vi "Action-x_control_excel.vi"() -> ()   [LabVIEW 2018, in "Report_modify.lvlib"]
uses:
  Report_modify.lvlib
panel:
  out "数据":string[][](array[string])
  in  "Excel._Worksheet":refnum<k7>
  in  "Excel._Application":refnum<k7>
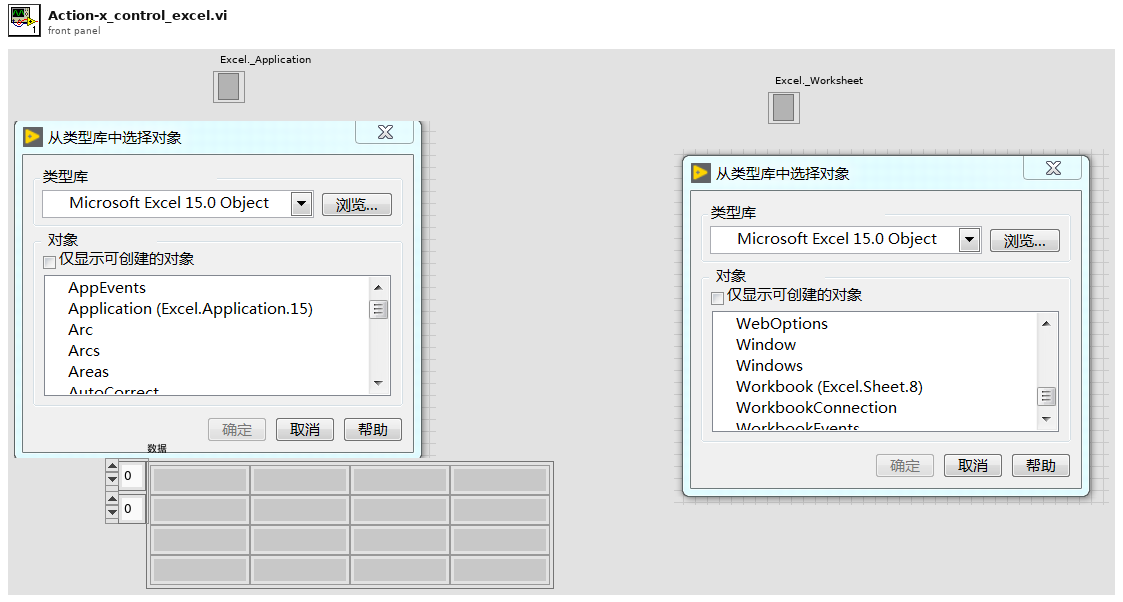
[diagram p1: front panel]
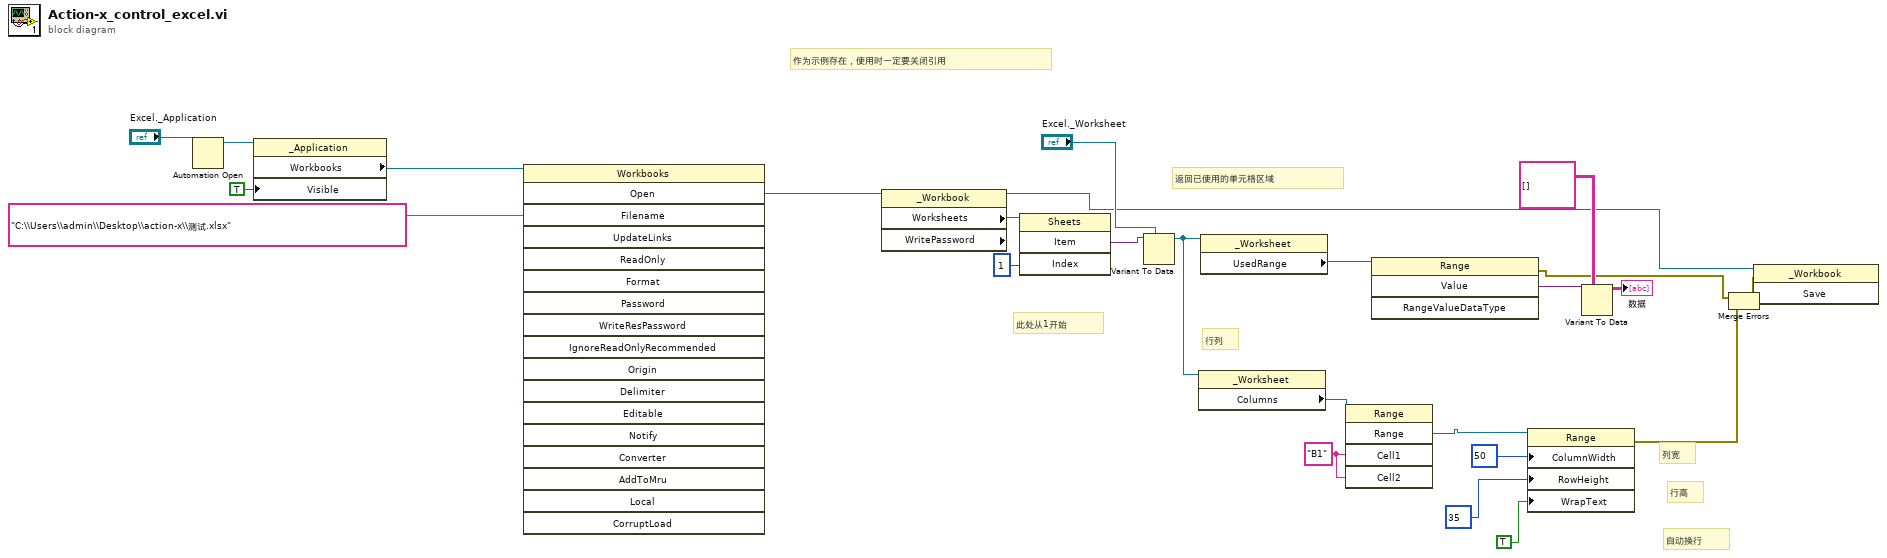
[diagram p0: block diagram]
diagram:
  w10 = "B1"
  # "作为示例存在，使用时一定要关闭引用"
  # "自动换行"
  # "行高"
  # "列宽"
  # "行列"
  # "返回已使用的单元格区域"
  # "此处从1开始"
  n1 = Automation Open(Automation Refnum="Excel._Application") -> (Automation Refnum=w24:refnum<k7>)  [unwired: 3 in, 1 out]
  n2 = property class="_Application"(reference=w24, "Visible"=TRUE) -> ("Workbooks"=w3:refnum<k7>)  [unwired: 1 in, 2 out]
  n3 = invoke class="Workbooks" method="Open"(reference=w3, "Filename"="C:\\Users\\admin\\Desktop\\action-x\\测试.xlsx") -> ("Open"=w23:refnum<k7>)  [unwired: 16 in, 17 out]
  n4 = property class="_Workbook" props=["Worksheets", "WritePassword"](reference=w23) -> (reference out=w8:refnum<k7>, "Worksheets"=w21:refnum<k7>)  [unwired: 1 in, 2 out]
  n5 = invoke class="Sheets" method="Item"(reference=w21, "Index"=1) -> ("Item"=w19:variant)  [unwired: 2 in, 3 out]
  n6 = Variant To Data(type="Excel._Worksheet", Variant=w19) -> (data=w13:refnum<k7>)  [unwired: 1 in, 1 out]
  n7 = property class="_Worksheet"(reference=w13) -> ("Columns"=w12:refnum<k7>)  [unwired: 1 in, 2 out]
  n8 = property class="_Worksheet"(reference=w13) -> ("UsedRange"=w17:refnum<k7>)  [unwired: 1 in, 2 out]
  n9 = invoke class="Range" method="Range"(reference=w12, "Cell1"=w10, "Cell2"=w10) -> ("Range"=w4:refnum<k7>)  [unwired: 2 in, 4 out]
  n10 = invoke class="Range" method="Value"(reference=w17) -> (error out=w5:errorcluster, "Value"=w16:variant)  [unwired: 3 in, 2 out]
  n11 = property class="Range"(reference=w4, "ColumnWidth"=50, "RowHeight"=35, "WrapText"=TRUE) -> (error out=w7:errorcluster)  [unwired: 1 in, 1 out]
  n12 = Variant To Data(type=string[][] [], Variant=w16) -> (data=→"数据":string[][])  [unwired: 1 in, 1 out]
  n13 = Merge Errors(w5, w7) -> (w6:errorcluster)
  n14 = invoke class="_Workbook" method="Save"(reference=w8, error in=w6) -> ()  [unwired: 1 in, 3 out]
